vi "OwnInterface20261013_ParentPath.vi"() -> ()   [LabVIEW 2024]
panel:
  out "error out":errorcluster caption="错误输出"
  out "Parent Path":path
  in  "Index":i32
  in  "Class Path":path
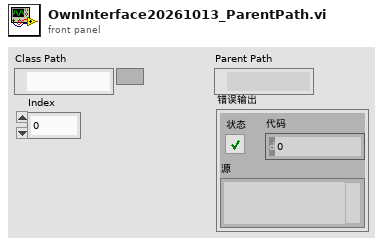
[diagram p1: front panel]
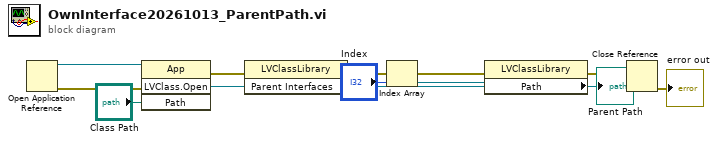
[diagram p0: block diagram]
diagram:
  n1 = Open Application Reference() -> (0:w10:errorcluster, 3:w12:refnum<vi>)  [unwired: 4 in]
  n2 = invoke class="App" method="LVClass.Open"(reference=w12, error in=w10, "Path"="Class Path") -> (error out=w8:errorcluster, "LVClass.Open"=w9:refnum<vi>)  [unwired: 1 in, 2 out]
  n3 = property class="LVClassLibrary"(reference=w9, error in=w8) -> (error out=w4:errorcluster, "Parent Interfaces"=w7:refnum<vi>[])  [unwired: 1 out]
  n4 = Index Array(array=w7, index="Index") -> (element=w5:refnum<vi>)
  n5 = property class="LVClassLibrary"(reference=w5, error in=w4) -> (error out=w2:errorcluster, "Path"=→"Parent Path":path)  [unwired: 1 out]
  n6 = Close Reference(reference=w9, error in (no error)=w2) -> (error out=→"error out":errorcluster)
